vi "Wait for TCP Ack.vi"(6 "options":T3={"ignore timeout error"=TRUE, "timeout ms (1000)"=1000}, 8 "error in (no error)":errorcluster, 10 "cmd name":string, 11 "connection info in":T1) -> (0 "error out":errorcluster, 1 "data string":string, 2 "timeout":bool, 3 "connection info out":T1)   [LabVIEW 2021, in "AudioGeneration.lvclass"]
uses:
  AudioGeneration.lvclass
  <vilib>/NI/STM/TCP/TCP Write Options.ctl
  <vilib>/NI/STM/TCP/TCP Connection Info.ctl
  <vilib>/NI/STM/SubVIs/MetaDataElement.ctl
  <vilib>/NI/STM/TCP/Read Message (TCP).vi
  AudioGeneration.lvclass/AudioGeneration.ctl
  <vilib>/NI/STM/NI STM.lvlib
  subVIs/utility/AudioGenUtility.lvlib
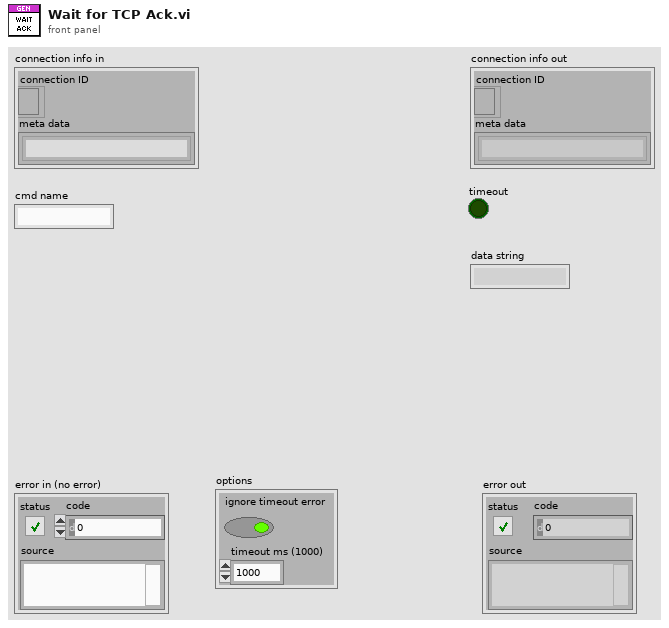
[diagram p1: front panel]
types:
  T1 = typedef "NI STM.lvlib/TCP Connection Info.ctl" = cluster{"connection ID":refnum<k5>, "meta data":T2[]}
  T2 = typedef "NI STM.lvlib/MetaDataElement.ctl" = string
  T3 = typedef "NI STM.lvlib/TCP Write Options.ctl" = cluster{"ignore timeout error":bool, "timeout ms (1000)":i32}
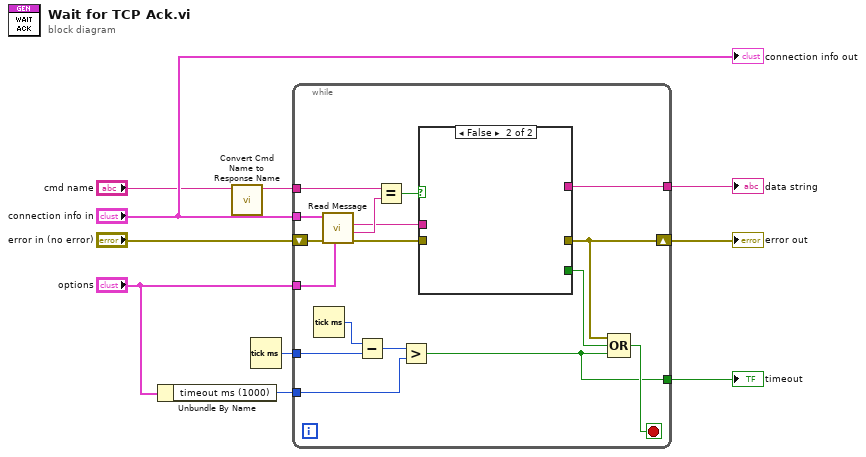
[diagram p0: block diagram]
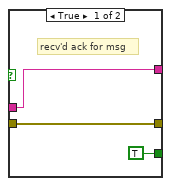
[diagram p2: hidden frame]
diagram:
  n1 = Unbundle By Name("options") -> ("timeout ms (1000)"=w9:i32)
  n2 = call "Convert Cmd Name to Response Name.vi"("cmd name"="cmd name") -> ("response name"=w2:string)  [unwired: 10 in]
  n3 = Tick Count (ms)() -> (millisecond timer value=w7:u32)
  n4 = while {
    tunnel: "connection info in" -> [w26]
    tunnel: w2 -> [w24]
    tunnel: "options" -> [w15]
    shift-right: [w19] -> w6
    shift-left: "error in (no error)" -> [w27]
    tunnel: w7 -> [w21]
    tunnel: w9 -> [w16]
    tunnel: [w14] -> w10
    tunnel: [w11] -> w1
    stop <- w17 stop-if-true
    n5 = Tick Count (ms)() -> (millisecond timer value=w22:u32)
    n6 = call-poly <vilib>:"Read Message.vi"("options"=w15, "error in"=w27, "connection info in"=w26) -> ("error out"=w25:errorcluster, "name"=w13:T2, "data string"=w12:string)  [unwired: 3 in, 3 out]
    n7 = Subtract(x=w22, y=w21) -> (x-y=w20:u32)
    n8 = Equal?(x=w24, y=w13) -> (x = y?=w23:bool)
    n9 = Greater?(x=w20, y=w16) -> (0:w14:bool)
    n10 = case shown="False" w23 {
      tunnel: w25 -> [w30 _]
      tunnel: [w30 _] -> w19
      tunnel: [TRUE _] -> w18
      tunnel: [w28 _] -> w11
      tunnel: w12 -> [w28 _]
      frame True {
        # "recv'd ack for msg"
      }
      frame False {
      }
    }
    n11 = Compound Arithmetic op=OR(w19, w18, w14) -> (w17:bool)
  }
  "timeout" <- w10
  "error out" <- w6
  "data string" <- w1
  "connection info out" <- "connection info in"
